vi "SC Quote Argument.vi"(9 "argument":string, 10 "windows?":bool) -> (1 "quoted argument":string)   [LabVIEW 2023]
doc: "Quotes one command-line argument for the shell that System Exec uses: double quotes for cmd.exe on Windows (a \" in the argument becomes ', since cmd has no escape for it), single quotes for sh elsewhere."
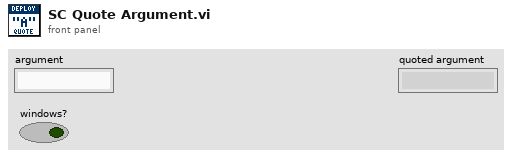
[diagram p1: front panel]
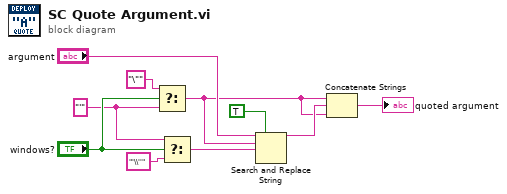
[diagram p0: block diagram]
diagram:
  w8 = "'"
  n1 = Select(t="\"", s="windows?", f=w8) -> (s? t:f=w2:string)
  n2 = Select(t=w8, s="windows?", f="'\\''") -> (s? t:f=w5:string)
  n3 = Search and Replace String(replace all?=TRUE, input string="argument", search string=w2, replace string=w5) -> (result string=w3:string)  [unwired: 4 in, 3 out]
  n4 = Concatenate Strings(w2, w3, w2) -> (→"quoted argument":string)
